vi "Module Init.vi"(8 "error in (no error)":errorcluster, 11 "GUI Manager Module in":refnum<class "GUI Manager Module.lvclass">) -> (0 "error out":errorcluster, 3 "GUI Manager Module out":refnum<class "GUI Manager Module.lvclass">)   [LabVIEW 2020, in "VolatusGUI.lvlib" / "GUI Manager Module.lvclass"]
uses:
  GUI Manager Module.lvclass
  C:/dev/lv20CE/relink/lv-volatus/Volatus/Module/Module.lvclass
  GUI Manager Module.lvclass/GUI Manager Module.ctl
  Volatus/Module/Module.lvclass/Module.ctl
  Volatus/MessageQ/MessageQ.lvclass/MessageQ.ctl
  Volatus/Module/Self Q.vi
  Volatus/MessageQ/Send.vi
  Volatus/Module/Module.lvclass
  lv-userprefs/User Prefs/PrefsDB/PrefsDB.lvclass
  lv-userprefs/User Prefs/Pref Group/Pref Group.lvclass
  C:/dev/lv20CE/relink/lv-volatus/VolatusGUI/GUI Manager Module/GUI Manager Module.lvclass
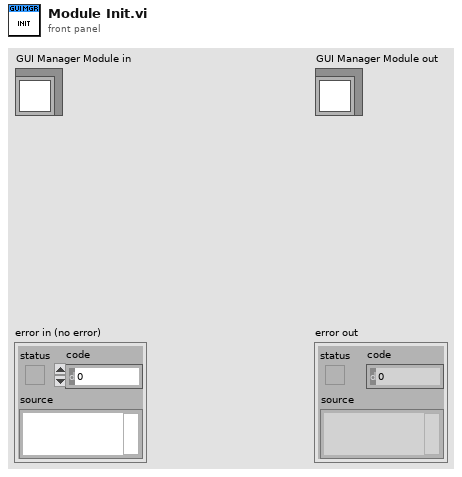
[diagram p1: front panel]
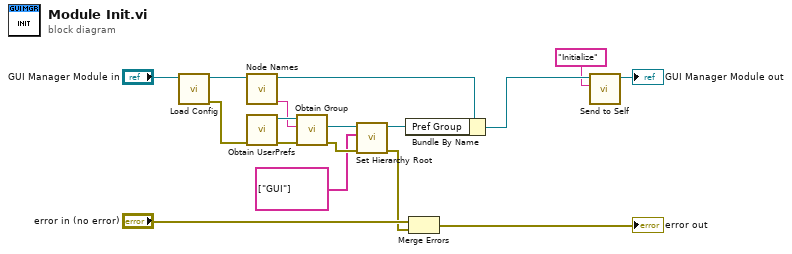
[diagram p0: block diagram]
diagram:
  n1 = call "Load Config.vi"("GUI Manager Module in"="GUI Manager Module in") -> ("error out"=w1:errorcluster, "GUI Manager Module out"=w2:refnum<class "GUI Manager Module.lvclass">)  [unwired: 9 in]
  n2 = call "Node Names.vi"("Module in"=w2) -> ("Node"=w11:string, "Module in"=w13:refnum<class "GUI Manager Module.lvclass">)  [unwired: 6 in, 3 out]
  n3 = call "Obtain UserPrefs.vi"("error in (no error)"=w1) -> ("error out"=w16:errorcluster, "PrefsDB out"=w12:refnum<class "PrefsDB.lvclass">)  [unwired: 9 in]
  n4 = call "Obtain Group.vi"("error in (no error)"=w16, "Group"=w11, "PrefsDB in (Singleton)"=w12) -> ("error out"=w17:errorcluster, "Pref Group"=w10:refnum<class "Pref Group.lvclass">)  [unwired: 6 in, 1 out]
  n5 = call "Set Hierarchy Root.vi"("error in (no error)"=w17, "Hierarchy Root"=string[] ["GUI"], "Pref Group in"=w10) -> ("error out"=w5:errorcluster, "Pref Group out"=w7:refnum<class "Pref Group.lvclass">)  [unwired: 7 in]
  n6 = Bundle By Name(cluster=w13, "Pref Group"=w7) -> (w8:refnum<class "GUI Manager Module.lvclass">)
  n7 = Merge Errors("error in (no error)", w5) -> (→"error out":errorcluster)
  n8 = call "Send to Self.vi"("Message ID"="Initialize", "Module in"=w8) -> ("Module in"=→"GUI Manager Module out":refnum<class "GUI Manager Module.lvclass">)  [unwired: 8 in, 1 out]
